vi "Configure.vi"(8 "error in (no error)":errorcluster, 9 "bit timing":T1, 10 "config":T2={"connection"={"host"="", "channel"=2, "cert path"=path "/home/lvuser/cansub_root_cert.crt"}, "bit rates"={"nominal bit rate"=500000, "nominal sample point"=80.0, "data bit rate"=2000000, "data sample point"=80.0}, "listen only"=FALSE, "filters"=[], "read mode"=enum."Poll", "max bytes per read"=4096, "reader FIFO depth"=0, "reader priority"=0, "ownership"=enum."Direct"} {"filters"."f2" format="%.0x"; "filters"."f1" format="%.0x"}, 11 "channel in":refnum<class "CANsub_Channel.lvclass">) -> (0 "error out":errorcluster, 3 "channel out":refnum<class "CANsub_Channel.lvclass">)   [LabVIEW 2021, in "CANsub_API.lvlib" / "CANsub_Channel.lvclass"]
doc: "Protected. Stores the config and the bit timing in the object; called only by Init. Must be overridden. Setup/teardown only: do not call in a periodic loop (allocates, may block)."
uses:
  CANsub_Channel.lvclass
  common/Typedefs/CANsub_connection.ctl
  common/CANsub_Common.lvlib
  common/Typedefs/CANsub_Bit_Rates.ctl
  Typedefs/CANsub_Filter.ctl
  CANsub_API.lvlib
  Typedefs/CANsub_Read_Mode.ctl
  Typedefs/CANsub_Ownership.ctl
  Typedefs/CANsub_Config.ctl
  common/Typedefs/Bit_Timing.ctl
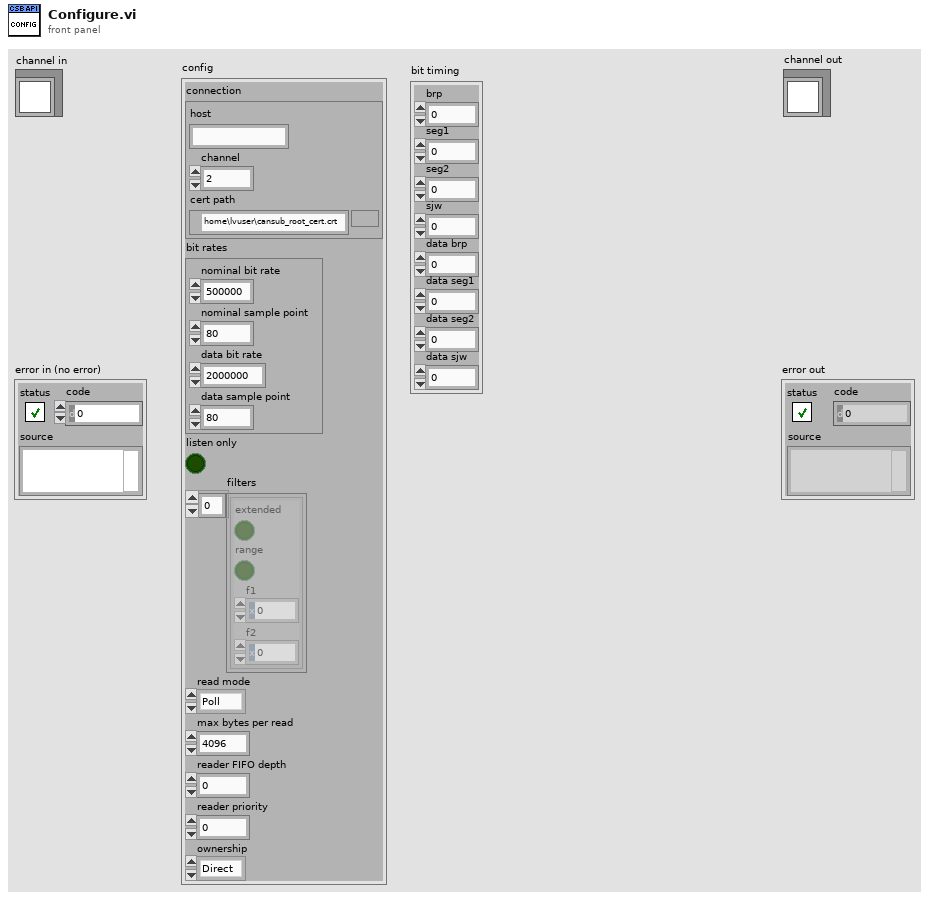
[diagram p1: front panel]
types:
  T1 = typedef "CANsub_Common.lvlib/Bit_Timing.ctl" = cluster{"brp":u16, "seg1":u16, "seg2":u16, "sjw":u16, "data brp":u16, "data seg1":u16, "data seg2":u16, "data sjw":u16}
  T2 = typedef "CANsub_API.lvlib/CANsub_Config.ctl" = cluster{"connection":T3, "bit rates":T4, "listen only":bool, "filters":T5[], "read mode":T6, "max bytes per read":i32, "reader FIFO depth":i32, "reader priority":i32, "ownership":T7}
  T3 = typedef "CANsub_Common.lvlib/CANsub_connection.ctl" = cluster{"host":string, "channel":u8, "cert path":path}
  T4 = typedef "CANsub_Common.lvlib/CANsub_Bit_Rates.ctl" = cluster{"nominal bit rate":u32, "nominal sample point":dbl, "data bit rate":u32, "data sample point":dbl}
  T5 = typedef "CANsub_API.lvlib/CANsub_Filter.ctl" = cluster{"extended":bool, "range":bool, "f1":u32, "f2":u32}
  T6 = typedef "CANsub_API.lvlib/CANsub_Read_Mode.ctl" = enum16{"Poll", "Reader"}
  T7 = typedef "CANsub_API.lvlib/CANsub_Ownership.ctl" = enum16{"Direct", "Shared"}
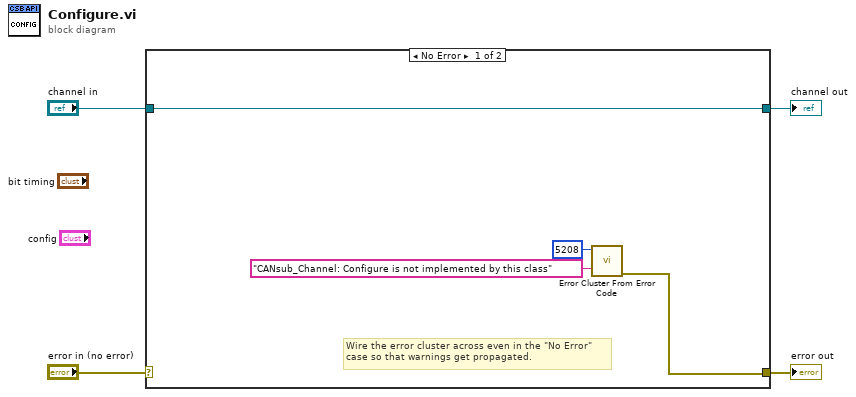
[diagram p0: block diagram]
diagram:
  n1 = case shown="No Error" "error in (no error)" {
    selector: "error in (no error)" -> [_ w10]
    tunnel: [w5 w10] -> w3
    tunnel: [w8 w9] -> w1
    tunnel: "channel in" -> [w8 w9]
    frame No Error {
      # "Wire the error cluster across even in the \"No Error\"\ncase so that warnings get propagated."
      n2 = call <vilib>:"Error Cluster From Error Code.vi"("error message (\"\")"="CANsub_Channel: Configure is not implemented by this class" ("error message (\"\")"), "error code (0)"=5208) -> ("error out"=w5:errorcluster)  [unwired: 7 in]
    }
    frame Error {
    }
  }
  "error out" <- w3
  "channel out" <- w1
